vi "Create PPL.vi"(0 "configuration":T1, 11 "error in":errorcluster) -> (15 "error out":errorcluster)   [LabVIEW 2021, in "InstrumentStudio Plug-In Editor.lvlib"]
uses:
  InstrumentStudio Plug-In Editor.lvlib
  <vilib>/AppBuilder/AB_API/PPL/NI_AB_API_PPL.lvclass
  Plugin Configuration.ctl
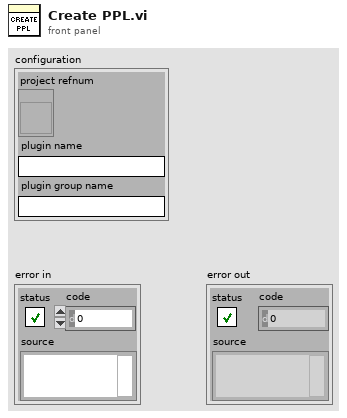
[diagram p1: front panel]
types:
  T1 = typedef "InstrumentStudio Plug-In Editor.lvlib/Plugin Configuration.ctl" = cluster{"project refnum":refnum<vi>, "plugin name":string, "plugin group name":string}
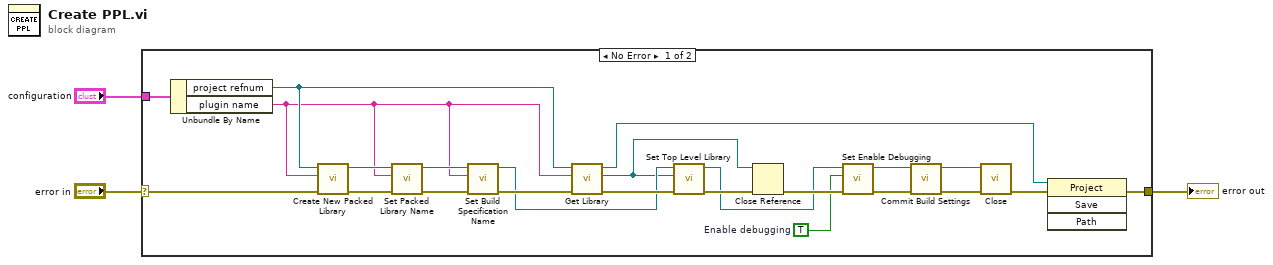
[diagram p0: block diagram]
diagram:
  n1 = case shown="No Error" "error in" {
    selector: "error in" -> [w19 w27]
    tunnel: "configuration" -> [w10 _]
    tunnel: [w4 w27] -> w1
    frame No Error {
      w9 = TRUE  # Enable debugging
      n2 = Unbundle By Name(w10) -> ("project refnum"=w12:refnum<vi>, "plugin name"=w11:string)
      n3 = call <vilib>:"Create New Packed Library.vi"("error in (no error)"=w19, "Build specification name"=w11, "Project Refnum"=w12) -> ("error out"=w23:errorcluster, "PPL out"=w22:refnum<class "NI_AB_API_PPL.lvclass">)  [unwired: 7 in]
      n4 = call-dynamic "Set Packed Library Name.vi"("error in (no error)"=w23, "Packed library name"=w11, "PPL in"=w22) -> ("error out"=w24:errorcluster, "PPL out"=w25:refnum<class "NI_AB_API_PPL.lvclass">)  [unwired: 7 in]
      n5 = call-dynamic "Set Build Specification Name.vi"("error in (no error)"=w24, "Build Specification Name"=w11, "NI_AB_API_PPL in"=w25) -> ("error out"=w18:errorcluster, "NI_AB_API_PPL out"=w14:refnum<class "NI_AB_API_PPL.lvclass">)  [unwired: 7 in]
      n6 = call "Get Library.vi"("error in"=w18, "library name"=w11, "project refnum in"=w12) -> ("error out"=w17:errorcluster, "library refnum"=w5:refnum<vi>, "project refnum out"=w6:refnum<vi>)  [unwired: 5 in, 1 out]
      n7 = call-dynamic "Set Top Level Library.vi"("error in (no error)"=w17, "ProjectItem Refnum"=w5, "PPL in"=w14) -> ("error out"=w16:errorcluster, "PPL out"=w13:refnum<class "NI_AB_API_PPL.lvclass">)  [unwired: 7 in]
      n8 = Close Reference(reference=w5, error in (no error)=w16) -> (error out=w15:errorcluster)
      n9 = call-dynamic "Set Enable Debugging.vi"("error in (no error)"=w15, "Enable debugging (false)"=w9, "PPL in"=w13) -> ("error out"=w21:errorcluster, "PPL out"=w20:refnum<class "NI_AB_API_PPL.lvclass">)  [unwired: 7 in]
      n10 = call-dynamic "Commit Build Settings.vi"("error in (no error)"=w21, "PPL in"=w20) -> ("error out"=w8:errorcluster, "PPL out"=w26:refnum<class "NI_AB_API_PPL.lvclass">)  [unwired: 8 in]
      n11 = call-dynamic "Close.vi"("error in (no error)"=w8, "DLL in"=w26) -> ("error out"=w7:errorcluster)  [unwired: 9 in]
      n12 = invoke class="Project" method="Save"(reference=w6, error in=w7) -> (error out=w4:errorcluster)  [unwired: 2 in, 3 out]
    }
    frame Error {
    }
  }
  "error out" <- w1
